vi "Get Run Mode.vi"(8 "error in (no error)":errorcluster caption="错误输入（无错误）", 11 "uRunMode":u32) -> (0 "error out":errorcluster caption="错误输出", 2 "function return":i32, 3 "uRunMode out":u32)   [LabVIEW 2017, in "smncsftmt.lvlib"]
doc: "__declspec(dllexport) int GetRunMode(unsigned int* uRunMode);"
uses:
  smncsftmt.lvlib
  smncsftmt.dll
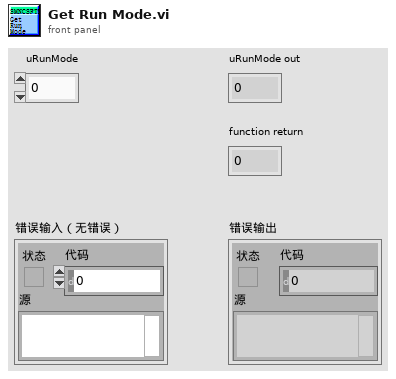
[diagram p1: front panel]
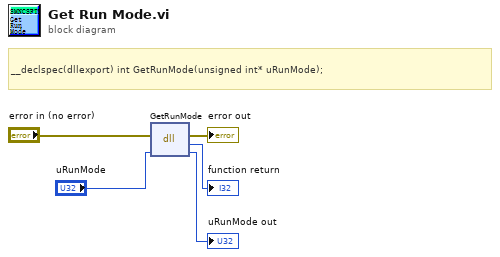
[diagram p0: block diagram]
diagram:
  # "__declspec(dllexport) int GetRunMode(unsigned int* uRunMode);"
  n1 = dll-call lib="PTH2oabs CUsersaDesktop\nLABVIEW范例National InstrumentsLabVIEW 2017user.lib\tsmncsftmtsmncsftmt.*" fn="GetRunMode"(error in="error in (no error)", "uRunMode"="uRunMode") -> (error out=→"error out":errorcluster, →"function return":i32, "uRunMode"=→"uRunMode out":u32)  [unwired: 2 in, 1 out]
